vi "Host.vi"() -> ()   [LabVIEW 2019]
uses:
  <vilib>/Bytelabs/ByteTCP/TCP_Class/TCP.lvclass
  TypeDef/TCPMessage.ctl
  <vilib>/Bytelabs/ByteChannelsSetting/ChannelSettingsLib/ChannelsRepos/ChannelsRepoXML/ChannelsRepoXML.lvclass
  TypeDef/listChannel.ctl
  TypeDef/ChannelInfo.ctl
  <vilib>/Bytelabs/ByteChannelsSetting/ChannelSettingsLib/ChannelsClasses/ChannelAnalog/AnalogIn/AnalogIn.lvclass
  ByteGSAPIBase/LimsTestStep/acquisitions.ctl
  ByteGSAPIBase/ByteGSAPIBase.lvclass
  <vilib>/Bytelabs/ByteChannelsSetting/ChannelSettingsLib/ChannelsClasses/ChannelBase/ChannelBase.lvclass
  ByteGSAPIBase/UpdateChannelsList/fields.ctl
  ByteGSAPIBase/TypeDef/Asset.ctl
  ByteGSAPIBase/TypeDef/StepAcquisition.ctl
panel:
  in  "Stop Multiple Log":bool
  out "Map":T1(c390)
  in  "Multiple Log":bool
  in  "Test":T2={"Step Id"=43, "Test Slug"="T0023", "Duration Seconds"=0.0, "Continous?"=FALSE}
  out "error out":errorcluster
  in  "Stop":bool
  out "Results":T3
  in  "Stop Sequence":bool
  out "Status":string
  out "Raws Readings":cluster{"tag":string, "Value":dbl}[](array[cluster])
  in  "Step  Request":bool
  in  "Channel List":T4[](array[typedef])
  in  "Load":bool
  in  "Configuration":bool
  out "Connected?":bool
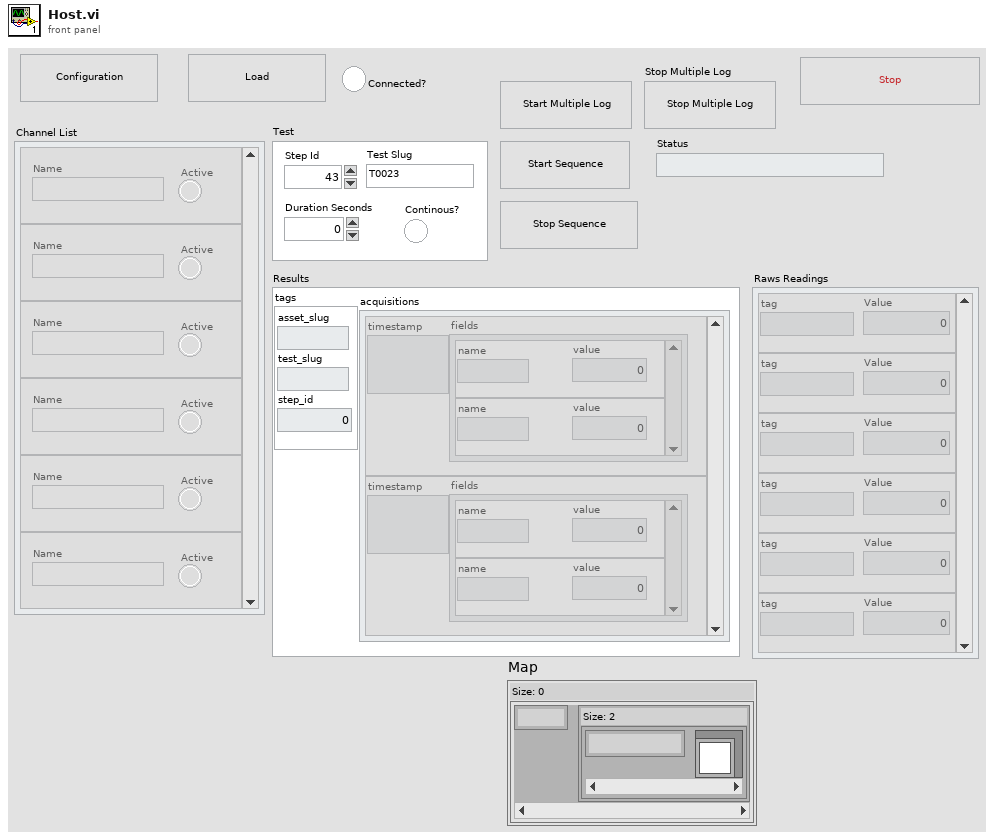
[diagram p1: front panel]
types:
  T1 = map{i32, map{string, refnum<class "ChannelBase.lvclass">}}
  T2 = cluster{"Step Id":u32, "Test Slug":string, "Duration Seconds":dbl, "Continous?":bool}
  T3 = typedef "ByteGSWebAPI.lvlib/ByteGSAPIBase.lvclass/acquisitions.ctl" = cluster{"tags":cluster{"step_id":i32, "test_slug":string, "asset_slug":string}, "acquisitions":cluster{"timestamp":string, "fields":cluster{"name":string, "value":dbl}[]}[]}
  T4 = typedef "listChannel.ctl" = cluster{"Name":string, "Active":bool}
  T5 = typedef "TCPMessage.ctl" = cluster{"Message":string, "Data":variant}
  T6 = cluster{"Event Registration Refnum":refnum<event-registration>, "ChannelsRepoBase out":refnum<class "ChannelsRepoXML.lvclass">, "TCP_Class":refnum<class "TCP.lvclass">, "Data":variant, "Stauts":string, "notifier out":refnum<notifier>}
  T7 = typedef "ChannelInfo.ctl" = cluster{"Tag":string, "HW Resource":string, "Raw":dbl}
  T8 = typedef "ByteGSWebAPI.lvlib/ByteGSAPIBase.lvclass/fields.ctl" = cluster{"asset_slug":string, "fields":string[]}
  T9 = cluster{"Channel List":T4[], "Test":cluster{"Step Id":u32, "Test Slug":string, "Duration Seconds":dbl, "Continous?":bool}}
  T10 = typedef "ByteGSWebAPI.lvlib/ByteGSAPIBase.lvclass/StepAcquisition.ctl" = cluster{"id":i32, "descrizione":string, "prova":cluster{"slug":string}, "assets":T11[], "criterio_accettazione":string, "valore_criterio_accettazione_max":dbl, "valore_criterio_accettazione_min":dbl, "udm_criterio_accettazione":string, "duration_prova":string, "udm_duration_prova":string, "valore_prova":dbl, "ordine":i32, "user":i32, "link_automation":string, "instruction_automation":string, "data_completamento_checklist":timestamp, "outcome":bool, "step_type":string, "channels":string[]}
  T11 = typedef "ByteGSWebAPI.lvlib/ByteGSAPIBase.lvclass/Asset.ctl" = cluster{"descrizione":string, "slug":string, "id":i32}
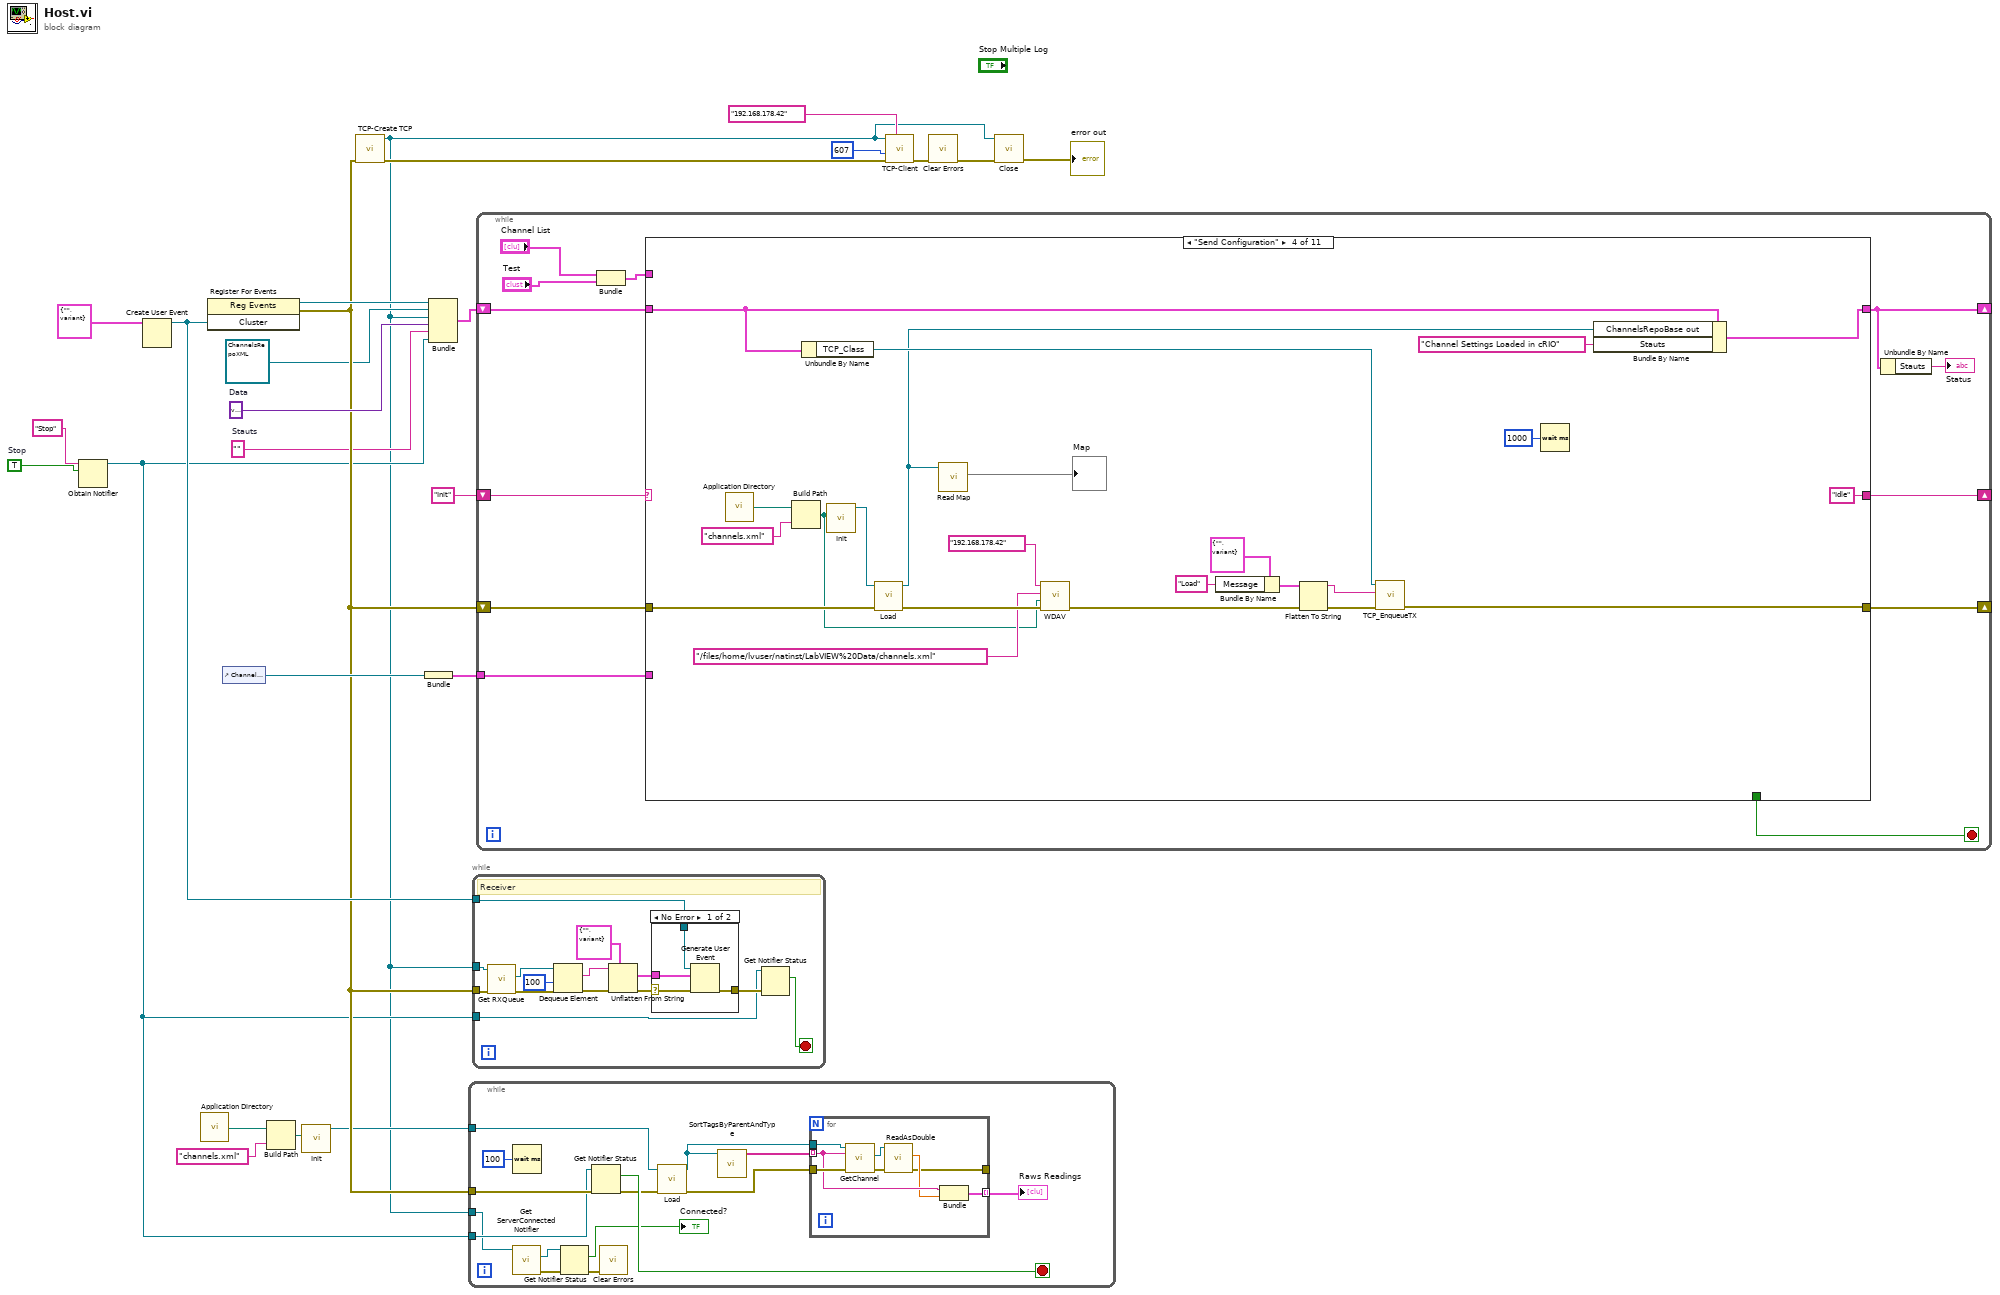
[diagram p0: block diagram]
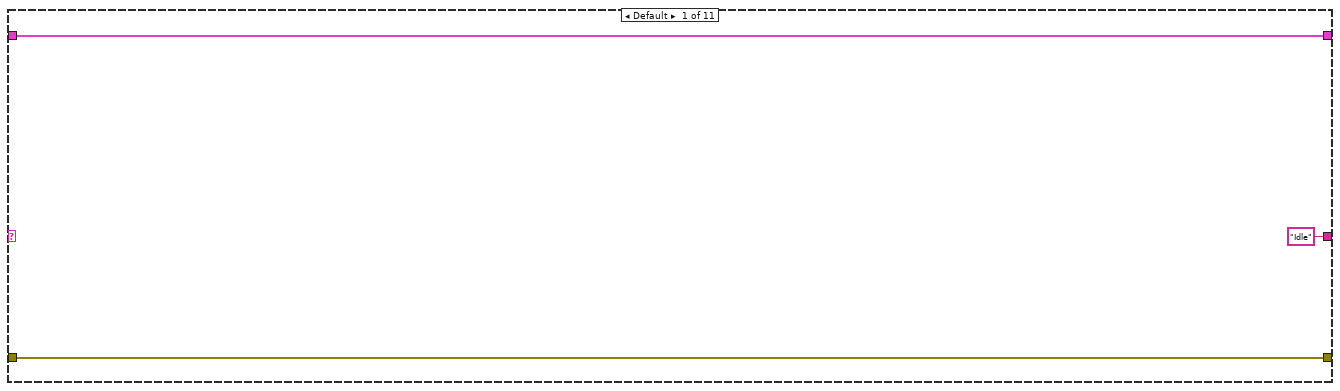
[diagram p2: hidden frame]
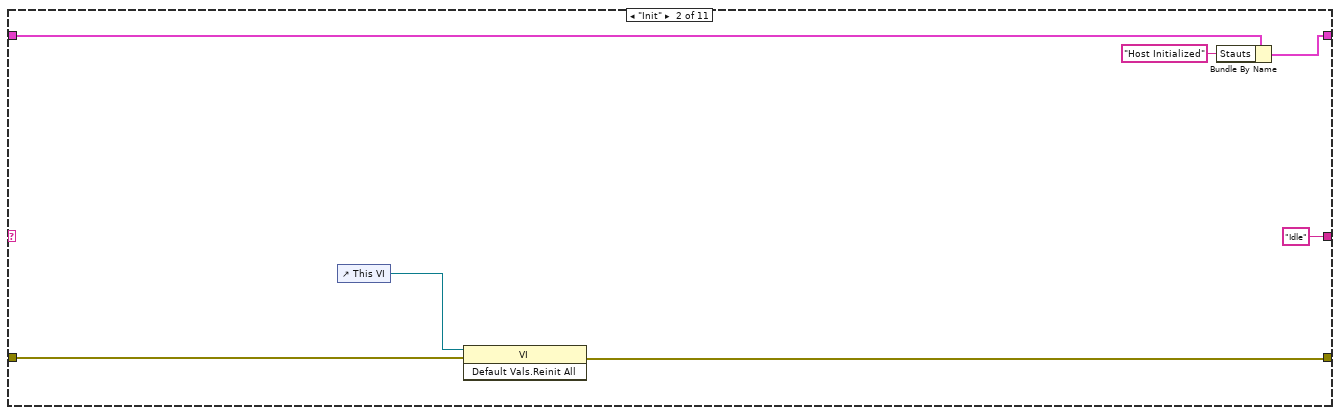
[diagram p3: hidden frame]
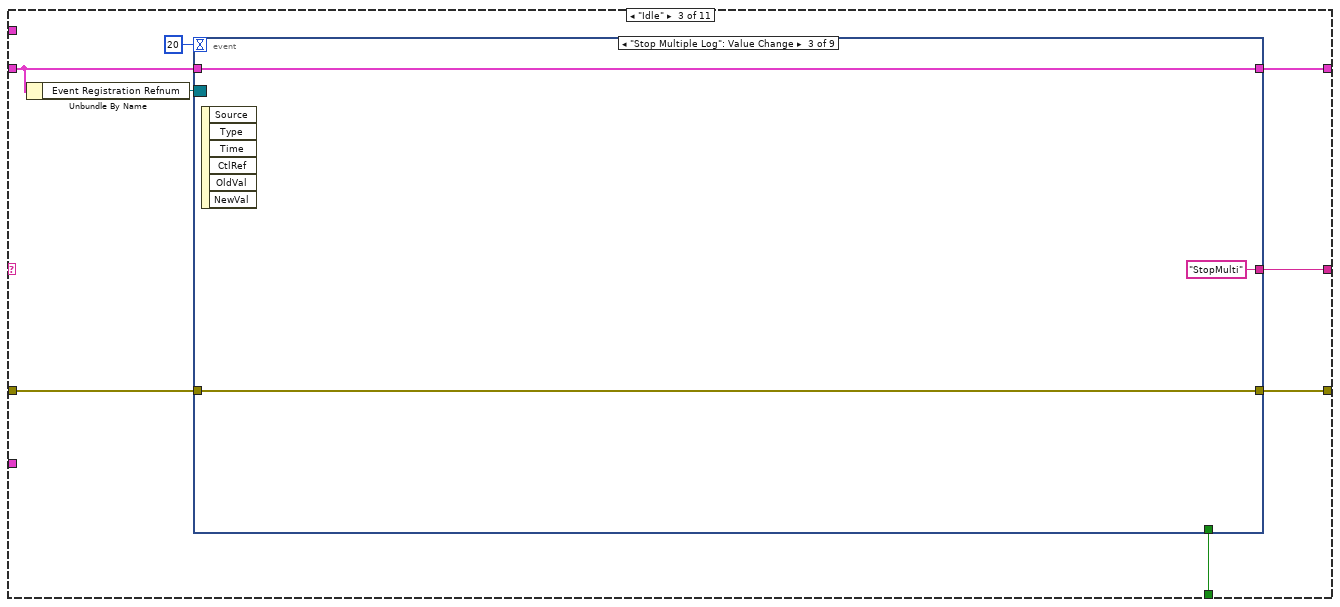
[diagram p4: hidden frame]
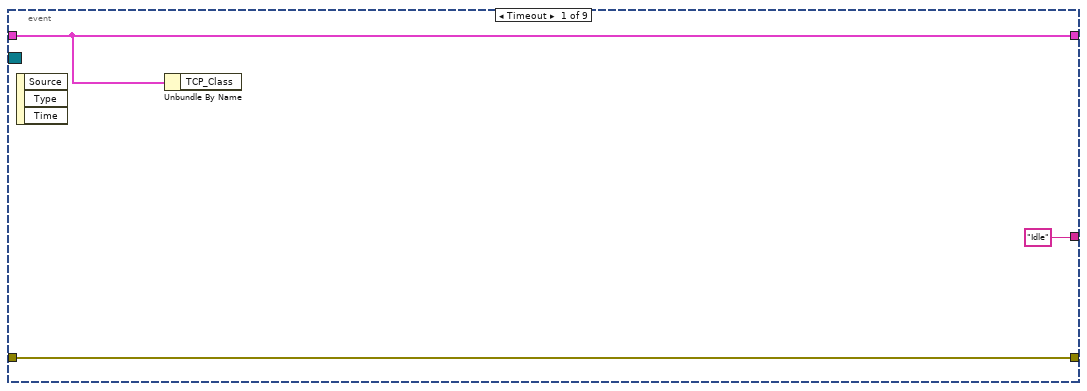
[diagram p5: hidden frame]
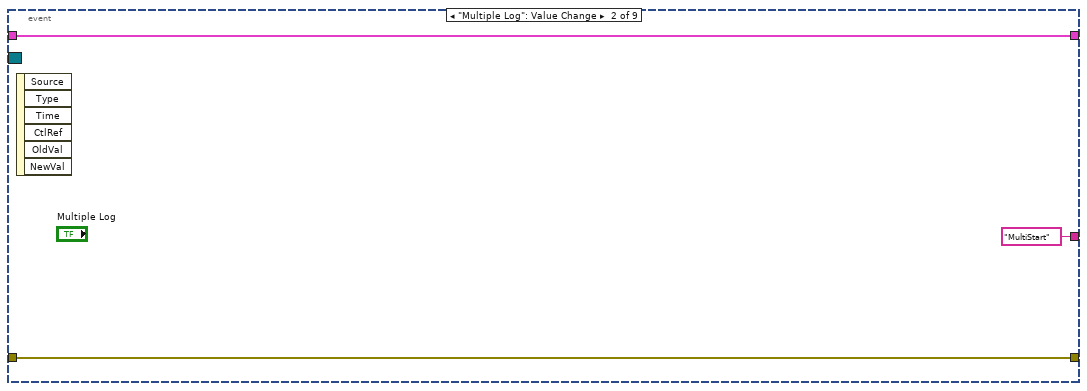
[diagram p6: hidden frame]
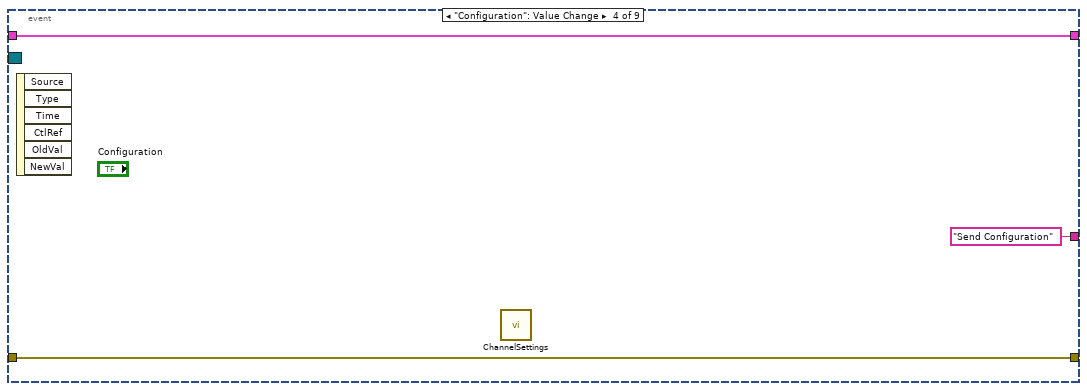
[diagram p7: hidden frame]
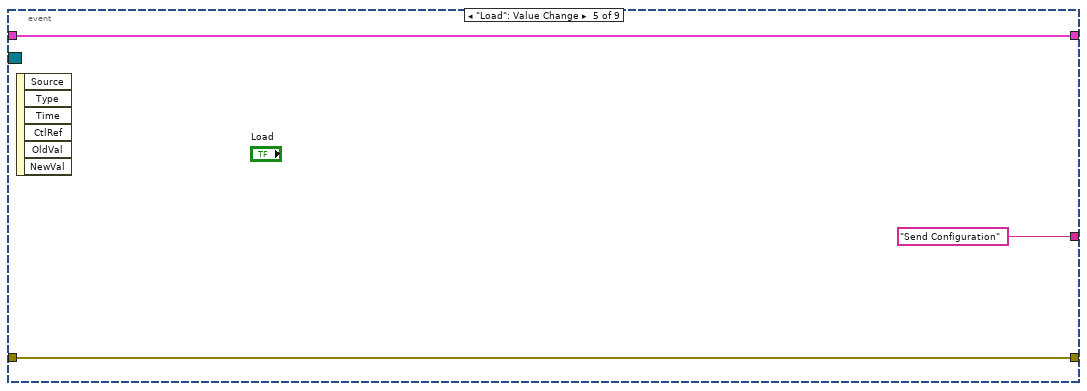
[diagram p8: hidden frame]
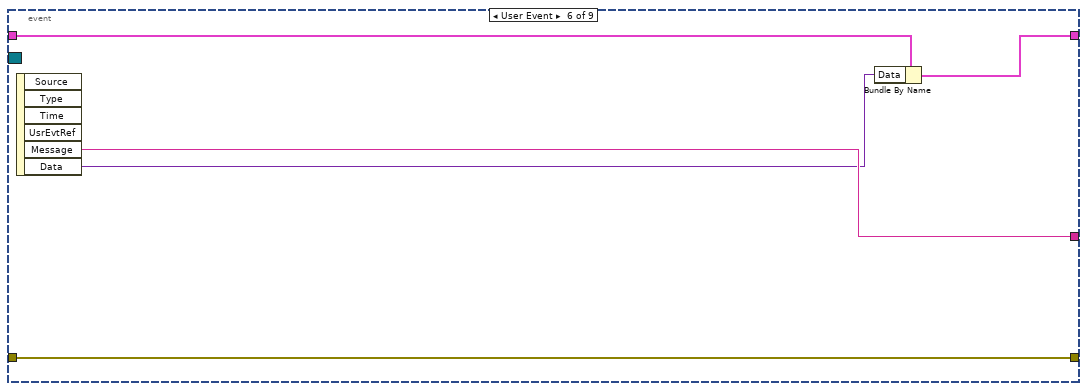
[diagram p9: hidden frame]
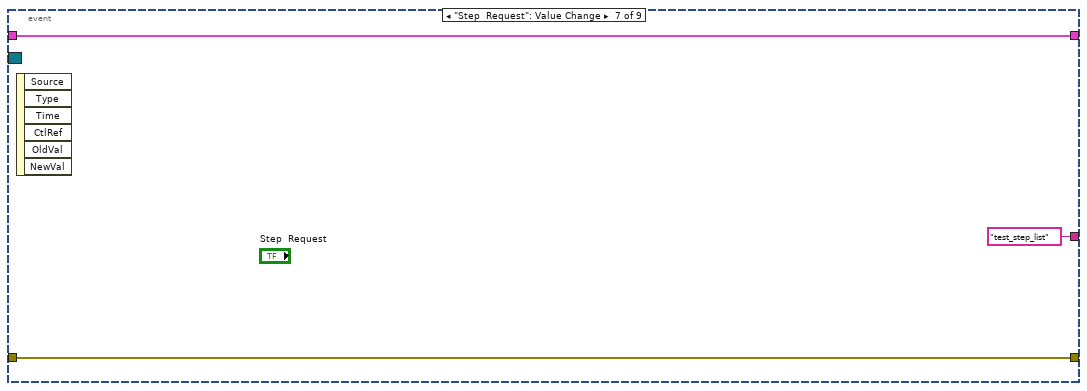
[diagram p10: hidden frame]
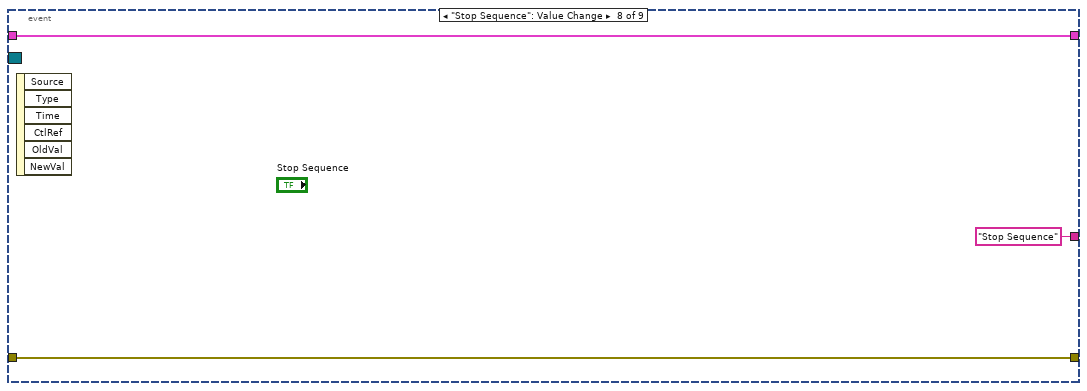
[diagram p11: hidden frame]
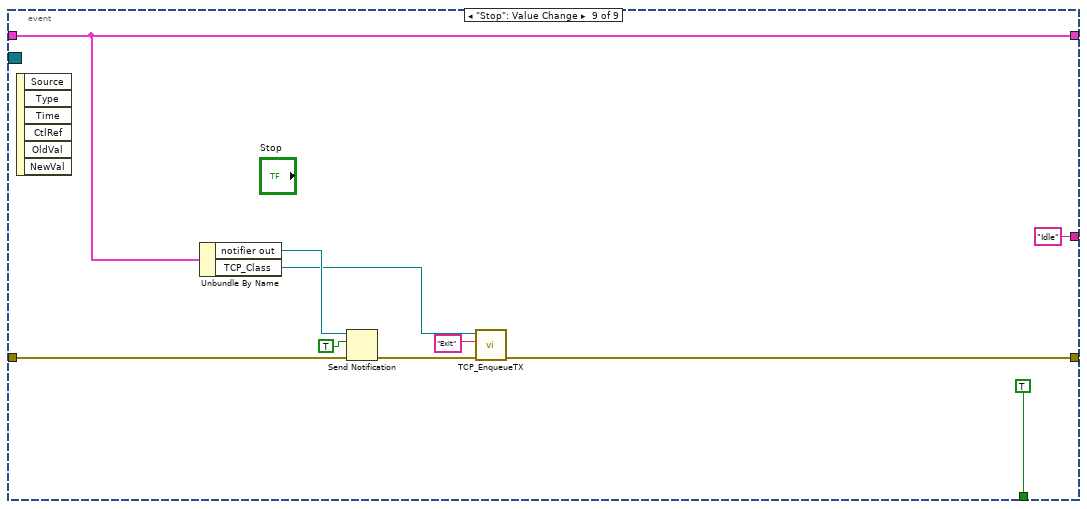
[diagram p12: hidden frame]
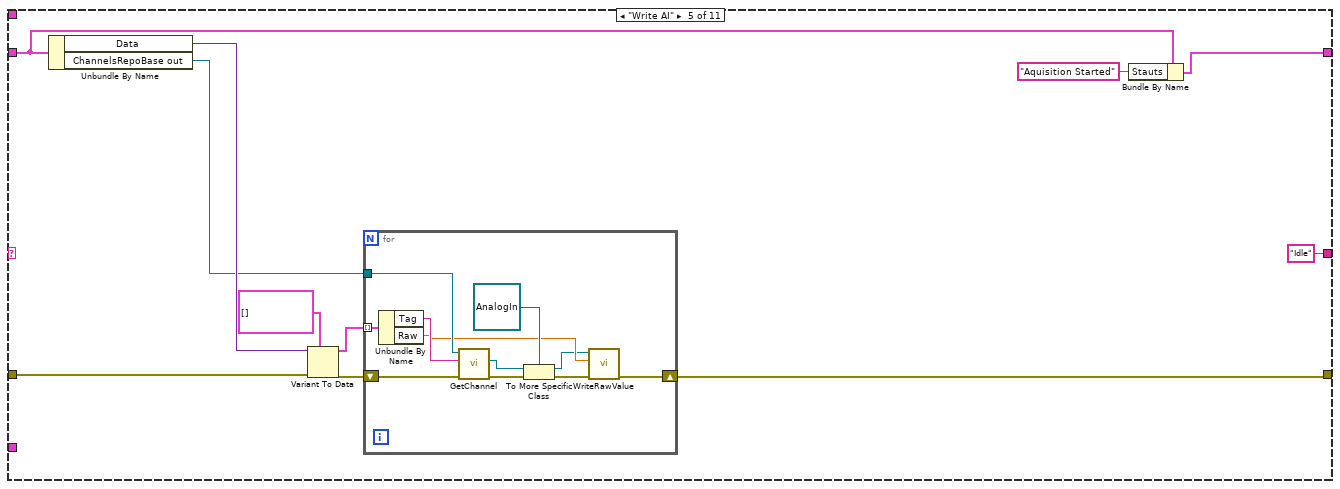
[diagram p13: hidden frame]
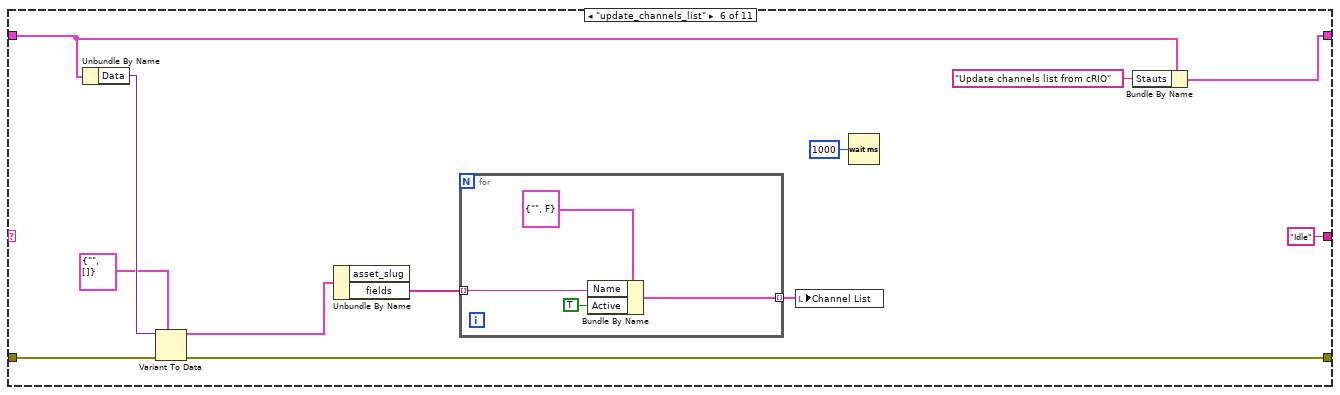
[diagram p14: hidden frame]
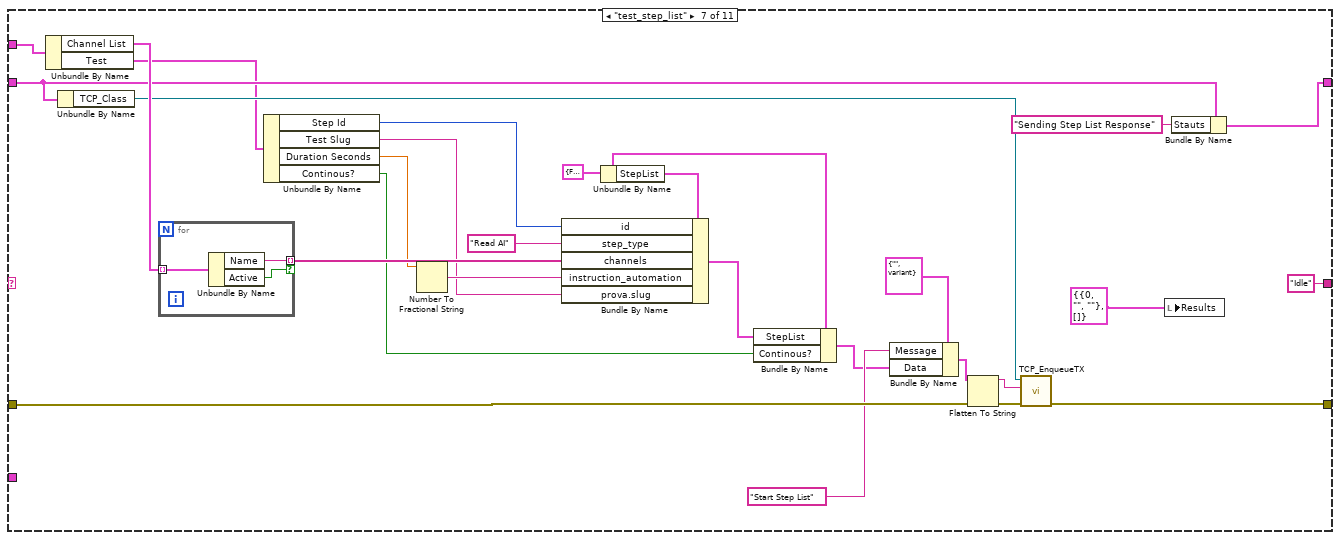
[diagram p15: hidden frame]
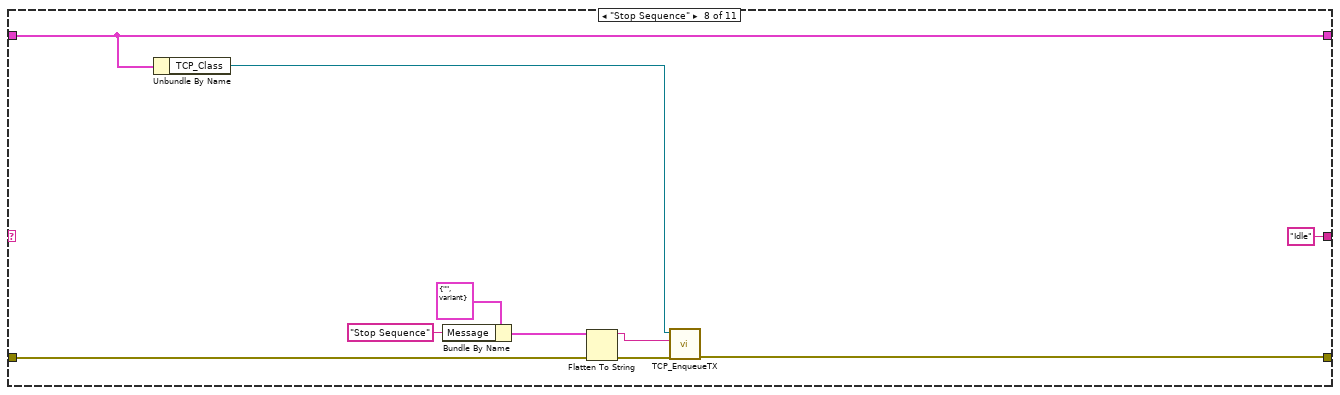
[diagram p16: hidden frame]
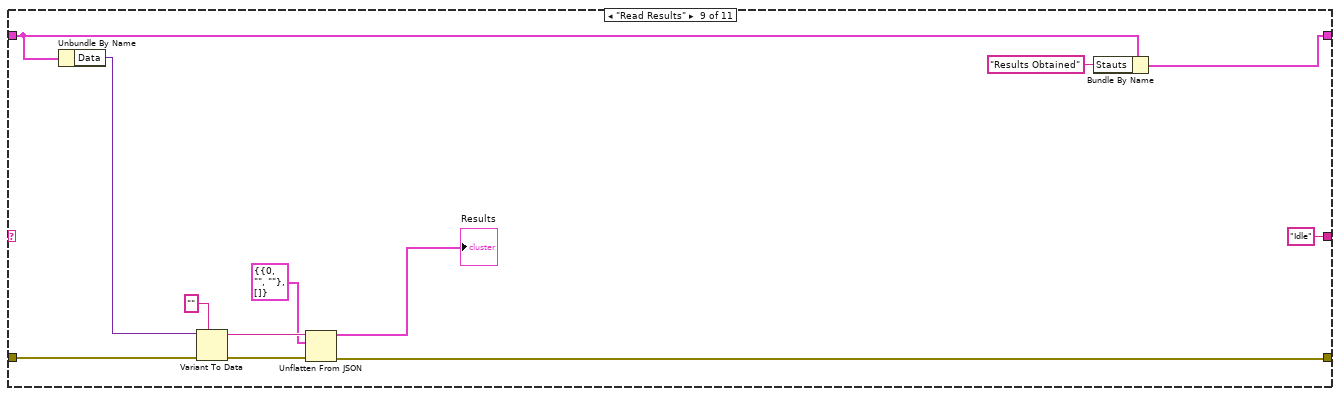
[diagram p17: hidden frame]
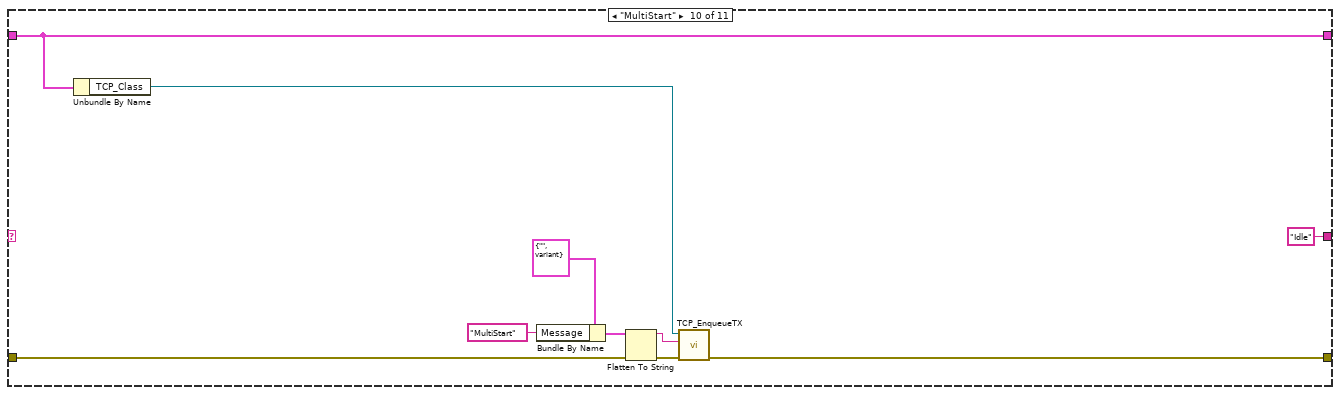
[diagram p18: hidden frame]
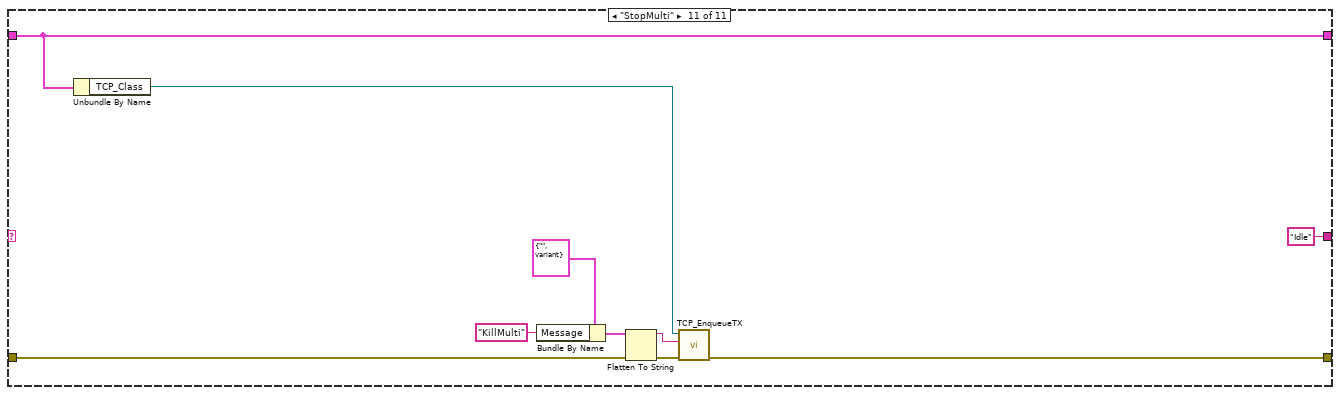
[diagram p19: hidden frame]
diagram:
  w11 = TRUE  # Stop
  w12 = ""  # Stauts
  w17 = variant  # Data
  n1 = Obtain Notifier(name (unnamed)="Stop", notification data type=w11) -> (notifier out=w9:refnum<notifier>)  [unwired: 2 in, 2 out]
  n2 = Create User Event(user event datatype=T5 {"Message"="", "Data"=variant} ("Cluster")) -> (user event=w22:refnum<user-event>)  [unwired: 1 in, 1 out]
  n3 = call <vilib>:"Application Directory.vi"() -> ("Application Directory"=w4:path)
  n4 = register-events(w22) -> (reference out=w21:refnum<event-registration>, error out=w14:errorcluster)  [unwired: 2 in]
  n5 = control-ref of="Channel List"() -> (w16:refnum<vi>)
  n6 = Build Path(base path=w4, name or relative path="channels.xml") -> (appended path=w5:path)
  n7 = call <vilib>:"Init.vi"("XML file path"=w5) -> ("ChannelsRepoXML out"=w2:refnum<class "ChannelsRepoXML.lvclass">)  [unwired: 10 in]
  n8 = call <vilib>:"TCP-Create TCP.vi"("error in (no error)"=w14) -> ("error out"=w23:errorcluster, "TCP_Class"=w1:refnum<class "TCP.lvclass">)  [unwired: 8 in, 1 out]
  n9 = Bundle("Channel List"=w16) -> (w15:cluster{"Channel List":refnum<vi>})  [unwired: 1 in]
  n10 = Bundle("Event Registration Refnum"=w21, "ChannelsRepoBase out"=refnum<class "ChannelsRepoXML.lvclass"> refnum, "TCP_Class"=w1, "Data"=w17, "Stauts"=w12, "notifier out"=w9) -> (w20:T6)  [unwired: 1 in]
  n11 = while {
    tunnel: w14 -> [w36]
    tunnel: w9 -> [w35]
    tunnel: w2 -> [w32]
    tunnel: w1 -> [w27]
    stop <- w34 stop-if-true
    n12 = call-dynamic "Get ServerConnectedNotifier.vi"("TCP in"=w27) -> ("error out"=w29:errorcluster, "IsServerConnected?"=w28:refnum<notifier>)  [unwired: 8 in, 1 out]
    n13 = Wait (ms)(milliseconds to wait=u32 100) -> ()  [unwired: 1 out]
    n14 = Get Notifier Status(notifier=w28, error in (no error)=w29) -> (current notification=→"Connected?":bool, error out=w30:errorcluster)  [unwired: 3 out]
    n15 = Get Notifier Status(notifier=w35, error in (no error)=w36) -> (current notification=w34:bool, error out=w33:errorcluster)  [unwired: 3 out]
    n16 = call <vilib>:"Clear Errors.vi"("error in (no error)"=w30) -> ()  [unwired: 5 in, 2 out]
    n17 = call <vilib>:"Load.vi"("error in (no error)"=w33, "ChannelsRepoBase in"=w32) -> ("error out"=w38:errorcluster, "ChannelsRepoBase out"=w37:refnum<class "ChannelsRepoXML.lvclass">)  [unwired: 7 in, 1 out]
    n18 = call <vilib>:"SortTagsByParentAndType.vi"("ChannelsRepoBase in"=w37) -> ("sorted tags"=w40:string[])  [unwired: 8 in, 2 out]
    n19 = for {
      tunnel: w38 -> [w48]
      tunnel: w40 -> [w45] mode=indexing
      tunnel: [w43] -> w39 mode=indexing
      tunnel: [w42] -> _
      tunnel: w37 -> [w41]
      n20 = call <vilib>:"GetChannel.vi"("error in (no error)"=w48, "tag"=w45, "ChannelsRepoBase in"=w41) -> ("error out"=w47:errorcluster, "channel"=w46:refnum<class "ChannelBase.lvclass">)  [unwired: 5 in, 2 out]
      n21 = call-dynamic "ReadAsDouble.vi"("error in (no error)"=w47, "ChannelBase in"=w46) -> ("error out"=w42:errorcluster, "Value"=w44:dbl)  [unwired: 7 in, 1 out]
      n22 = Bundle("tag"=w45, "Value"=w44) -> (w43:cluster{"tag":string, "Value":dbl})  [unwired: 1 in]
    }
    "Raws Readings" <- w39
  }
  n23 = while {
    tunnel: w1 -> [w57]
    tunnel: w14 -> [w58]
    tunnel: w22 -> [w61]
    tunnel: w9 -> [w51]
    stop <- w50 stop-if-true
    # "Receiver"
    n24 = call-dynamic "Get RXQueue.vi"("error in (no error)"=w58, "TCP in"=w57) -> ("error out"=w56:errorcluster, "RX"=w53:refnum<queue>)  [unwired: 7 in, 1 out]
    n25 = Dequeue Element(queue=w53, timeout in ms (-1)=100, error in (no error)=w56) -> (element=w54:string, error out=w55:errorcluster)  [unwired: 2 out]
    n26 = Unflatten From String(type=T5 {"Message"="", "Data"=variant} ("Cluster"), binary string=w54, error in (no error)=w55) -> (value=w60:T5, error out=w62:errorcluster)  [unwired: 2 in, 1 out]
    n27 = case shown="No Error" w62 {
      selector: w62 -> [w66 _]
      tunnel: w61 -> [w65 _]
      tunnel: w60 -> [w64 _]
      tunnel: [w63 _] -> w52
      frame No Error {
        n28 = Generate User Event(user event=w65, event data cluster=w64, error in=w66) -> (error out=w63:errorcluster)  [unwired: 1 in, 1 out]
      }
      frame Error {
      }
    }
    n29 = Get Notifier Status(notifier=w51, error in (no error)=w52) -> (current notification=w50:bool)  [unwired: 4 out]
  }
  n30 = while {
    shift-right: [w70] -> _
    shift-left: w20 -> [w76]
    shift-right: [w77] -> _
    shift-left: "Init" -> [w78]
    shift-right: [w74] -> _
    shift-left: w14 -> [w75]
    tunnel: w15 -> [w71]
    stop <- w68 stop-if-true
    n31 = Bundle("Channel List"="Channel List", "Test"="Test") -> (w72:T9)  [unwired: 1 in]
    n32 = case shown="\"Send Configuration\"" w78 {
      tunnel: ["Idle" "Idle" w93 "Idle" "Idle" ("Message") "Idle" ("Message") "Idle" ("Message") "Idle" ("Message") "Idle" ("Message") "Idle" ("Message") "Idle" ("Message")] -> w77
      tunnel: w76 -> [w81 w84 w91 w147 w158 w182 w207 w225 w238 w254 w264]
      tunnel: [w81 w82 w92 w146 w157 w180 w206 w225 w236 w254 w264] -> w70
      tunnel: w75 -> [w79 w87 w95 w148 w161 w189 w220 w228 w242 w249 w259]
      tunnel: [w79 w85 w94 w144 w160 w184 w210 w227 w241 w248 w258] -> w74
      tunnel: w72 -> [_ _ _ _ _ _ w218 _ _ _ _]
      tunnel: w71 -> [_ _ _ _ _ _ _ _ _ _ _]
      tunnel: [_ _ w89 _ _ _ _ _ _ _ _] -> w68
      frame Default {
      }
      frame "Init" {
        n33 = control-ref of="This VI"() -> (w86:refnum<vi>)
        n34 = invoke class="VI" method="Default Vals.Reinit All"(reference=w86, error in=w87) -> (error out=w85:errorcluster)  [unwired: 1 in, 2 out]
        n35 = Bundle By Name(cluster=w84, "Stauts"="Host Initialized") -> (w82:T6)
      }
      frame "Idle" {
        n36 = Unbundle By Name(w91) -> ("Event Registration Refnum"=w90:refnum<event-registration>)
        n37 = event shown="[2] \"Stop Multiple Log\": Value Change" {
          selector: w90 -> [_ _ _ _ _ _ _ _ _]
          dyn-events: _ -> [_ _ _ _ _ _ _ _ _]
          timeout: 20 -> [_ _ _ _ _ _ _ _ _]
          tunnel: w91 -> [w98 w102 w105 w108 w111 w115 w119 w121 w130]
          tunnel: w95 -> [w97 w101 w104 w107 w109 w112 w118 w122 w128]
          tunnel: [w97 w101 w104 w107 w109 w112 w118 w122 w125] -> w94
          tunnel: ["Idle" "MultiStart" ("Message") "StopMulti" ("Message") "Send Configuration" "Send Configuration" w116 "test_step_list" ("Message") "Stop Sequence" ("Message") "Idle" ("Message")] -> w93
          tunnel: [w98 w102 w105 w108 w111 w114 w119 w121 w130] -> w92
          tunnel: [_ _ _ _ _ _ _ _ TRUE] -> w89
          event Timeout {
            n38 = event-data() -> ()  [unwired: 1 in, 3 out]
            n39 = Unbundle By Name(w98) -> ()  [unwired: 1 out]
          }
          event "Multiple Log": Value Change {
            n40 = event-data() -> ()  [unwired: 1 in, 6 out]
          }
          event "Stop Multiple Log": Value Change {
            n41 = event-data() -> ()  [unwired: 1 in, 6 out]
          }
          event "Configuration": Value Change {
            n42 = event-data() -> ()  [unwired: 1 in, 6 out]
            n43 = call "ChannelSettings.vi"() -> ()  [unwired: 12 in]
          }
          event "Load": Value Change {
            n44 = event-data() -> ()  [unwired: 1 in, 6 out]
          }
          event User Event {
            n45 = event-data() -> ("Message"=w116:string, "Data"=w113:variant)  [unwired: 1 in, 4 out]
            n46 = Bundle By Name(cluster=w115, "Data"=w113) -> (w114:T6)
          }
          event "Step  Request": Value Change {
            n47 = event-data() -> ()  [unwired: 1 in, 6 out]
          }
          event "Stop Sequence": Value Change {
            n48 = event-data() -> ()  [unwired: 1 in, 6 out]
          }
          event "Stop": Value Change {
            n49 = event-data() -> ()  [unwired: 1 in, 6 out]
            n50 = Unbundle By Name(w130) -> ("notifier out"=w129:refnum<notifier>, "TCP_Class"=w124:refnum<class "TCP.lvclass">)
            n51 = Send Notification(notification=TRUE, notifier=w129, error in (no error)=w128) -> (error out=w126:errorcluster)  [unwired: 1 out]
            n52 = call-dynamic "TCP_EnqueueTX.vi"("error in (no error)"=w126, "Msg to Transmit"="Exit", "TCP in"=w124) -> ("error out"=w125:errorcluster)  [unwired: 7 in, 1 out]
          }
        }
      }
      frame "Send Configuration" {
        n53 = call <vilib>:"Application Directory.vi"() -> ("Application Directory"=w151:path)
        n54 = Build Path(base path=w151, name or relative path="channels.xml") -> (appended path=w135:path)
        n55 = Unbundle By Name(w147) -> ("TCP_Class"=w143:refnum<class "TCP.lvclass">)
        n56 = call <vilib>:"Init.vi"("XML file path"=w135) -> ("ChannelsRepoXML out"=w150:refnum<class "ChannelsRepoXML.lvclass">)  [unwired: 10 in]
        n57 = call <vilib>:"Load.vi"("error in (no error)"=w148, "ChannelsRepoBase in"=w150) -> ("error out"=w139:errorcluster, "ChannelsRepoBase out"=w134:refnum<class "ChannelsRepoXML.lvclass">)  [unwired: 7 in, 1 out]
        n58 = call <vilib>:"Read Map.vi"("ChannelsRepoBase in"=w134) -> ("Map"=→"Map":T1)  [unwired: 9 in, 1 out]
        n59 = call "WDAV.vi"("error in (no error)"=w139, "local file path"=w135, "remote path with slash files"="/files/home/lvuser/natinst/LabVIEW%20Data/channels.xml" ("string"), "target ip"="192.168.178.42") -> ("error out"=w138:errorcluster)  [unwired: 7 in]
        n60 = Bundle By Name(cluster=T5 {"Message"="", "Data"=variant} ("Cluster"), "Message"="Load") -> (w152:T5)
        n61 = Flatten To String(anything=w152, error in (no error)=w138) -> (data string=w142:string, error out=w145:errorcluster)  [unwired: 2 in, 1 out]
        n62 = call-dynamic "TCP_EnqueueTX.vi"("error in (no error)"=w145, "Msg to Transmit"=w142, "TCP in"=w143) -> ("error out"=w144:errorcluster)  [unwired: 7 in, 1 out]
        n63 = Wait (ms)(milliseconds to wait=u32 1000) -> ()  [unwired: 1 out]
        n64 = Bundle By Name(cluster=w147, "ChannelsRepoBase out"=w134, "Stauts"="Channel Settings Loaded in cRIO") -> (w146:T6)
      }
      frame "Write AI" {
        n65 = Unbundle By Name(w158) -> ("Data"=w166:variant, "ChannelsRepoBase out"=w163:refnum<class "ChannelsRepoXML.lvclass">)
        n66 = Variant To Data(error in=w161, type=T7[] [] ("Array"), Variant=w166) -> (data=w162:T7[], error out=w164:errorcluster)
        n67 = for {
          tunnel: w163 -> [w175]
          shift-right: [w169] -> w160
          shift-left: w164 -> [w177]
          tunnel: w162 -> [w167] mode=indexing
          n68 = Unbundle By Name(w167) -> ("Tag"=w176:string, "Raw"=w171:dbl)
          n69 = call <vilib>:"GetChannel.vi"("error in (no error)"=w177, "tag"=w176, "ChannelsRepoBase in"=w175) -> ("error out"=w174:errorcluster, "channel"=w168:refnum<class "ChannelBase.lvclass">)  [unwired: 5 in, 2 out]
          n70 = To More Specific Class(target class=refnum<class "AnalogIn.lvclass"> refnum ("ChannelSettings.lvlib:ChannelsClasses.lvlib:AnalogIn.lvclass"), reference=w168, error in=w174) -> (specific class reference=w170:refnum<class "AnalogIn.lvclass">, error out=w172:errorcluster)
          n71 = call <vilib>:"WriteRawValue.vi"("error in (no error)"=w172, "Raw value"=w171, "AnalogIn in"=w170) -> ("error out"=w169:errorcluster)  [unwired: 7 in, 1 out]
        }
        n72 = Bundle By Name(cluster=w158, "Stauts"="Aquisition Started") -> (w157:T6)
      }
      frame "update_channels_list" {
        n73 = Unbundle By Name(w182) -> ("Data"=w188:variant)
        n74 = Variant To Data(error in=w189, type=T8 {"asset_slug"="", "fields"=[]} ("Channels"), Variant=w188) -> (data=w183:T8, error out=w184:errorcluster)
        n75 = Unbundle By Name(w183) -> ("fields"=w186:string[])  [unwired: 1 out]
        n76 = for {
          tunnel: w186 -> [w192] mode=indexing
          tunnel: [w190] -> w185 mode=indexing
          n77 = Bundle By Name(cluster=T4 {"Name"="", "Active"=FALSE} ("Cluster"), "Name"=w192, "Active"=TRUE) -> (w190:T4)
        }
        n78 = local write "Channel List"(w185) -> ()
        n79 = Wait (ms)(milliseconds to wait=u32 1000) -> ()  [unwired: 1 out]
        n80 = Bundle By Name(cluster=w182, "Stauts"="Update channels list from cRIO") -> (w180:T6)
      }
      frame "test_step_list" {
        w197 = cluster{"Continous?":bool, "StepList":T10} {"Continous?"=FALSE, "StepList"={"id"=0, "descrizione"="", "prova"={"slug"=""}, "assets"=[], "criterio_accettazione"="", "valore_criterio_accettazione_max"=0.0, "valore_criterio_accettazione_min"=0.0, "udm_criterio_accettazione"="", "duration_prova"="", "udm_duration_prova"="", "valore_prova"=0.0, "ordine"=0, "user"=0, "link_automation"="", "instruction_automation"="", "data_completamento_checklist"=timestamp(0 s since 1904-01-01), "outcome"=FALSE, "step_type"="", "channels"=[]}}
        n81 = Unbundle By Name(w218) -> ("Channel List"=w217:T4[], "Test"=w200:T2)
        n82 = Unbundle By Name(w207) -> ("TCP_Class"=w209:refnum<class "TCP.lvclass">)
        n83 = for {
          tunnel: w217 -> [w223] mode=indexing
          tunnel: [w222] -> w216 mode=indexing if=w221
          n84 = Unbundle By Name(w223) -> ("Name"=w222:string, "Active"=w221:bool)
        }
        n85 = Unbundle By Name(w200) -> ("Step Id"=w202:u32, "Test Slug"=w201:string, "Duration Seconds"=w199:dbl, "Continous?"=w195:bool)
        n86 = Number To Fractional String(number=w199) -> (F-format string=w204:string)  [unwired: 3 in]
        n87 = Unbundle By Name(w197) -> ("StepList"=w198:T10)
        n88 = Bundle By Name(cluster=w198, "id"=w202, "step_type"="Read AI", "channels"=w216, "instruction_automation"=w204, "prova.slug"=w201) -> (w196:T10)
        n89 = Bundle By Name(cluster=w197, "StepList"=w196, "Continous?"=w195) -> (w194:cluster{"Continous?":bool, "StepList":T10})
        n90 = Bundle By Name(cluster=T5 {"Message"="", "Data"=variant} ("Cluster"), "Message"="Start Step List", "Data"=w194) -> (w212:T5)
        n91 = Flatten To String(anything=w212, error in (no error)=w220) -> (data string=w211:string, error out=w213:errorcluster)  [unwired: 2 in, 1 out]
        n92 = call-dynamic "TCP_EnqueueTX.vi"("error in (no error)"=w213, "Msg to Transmit"=w211, "TCP in"=w209) -> ("error out"=w210:errorcluster)  [unwired: 7 in, 1 out]
        n93 = local write "Results"(T3 {"tags"={"step_id"=0, "test_slug"="", "asset_slug"=""}, "acquisitions"=[]}) -> ()
        n94 = Bundle By Name(cluster=w207, "Stauts"="Sending Step List Response") -> (w206:T6)
      }
      frame "Stop Sequence" {
        n95 = Unbundle By Name(w225) -> ("TCP_Class"=w224:refnum<class "TCP.lvclass">)
        n96 = Bundle By Name(cluster=T5 {"Message"="", "Data"=variant} ("Cluster"), "Message"="Stop Sequence") -> (w231:T5)
        n97 = Flatten To String(anything=w231, error in (no error)=w228) -> (data string=w229:string, error out=w230:errorcluster)  [unwired: 2 in, 1 out]
        n98 = call-dynamic "TCP_EnqueueTX.vi"("error in (no error)"=w230, "Msg to Transmit"=w229, "TCP in"=w224) -> ("error out"=w227:errorcluster)  [unwired: 7 in, 1 out]
      }
      frame "Read Results" {
        n99 = Unbundle By Name(w238) -> ("Data"=w240:variant)
        n100 = Variant To Data(error in=w242, type="", Variant=w240) -> (data=w243:string, error out=w245:errorcluster)
        n101 = Unflatten From JSON(JSON string=w243, type and defaults=T3 {"tags"={"step_id"=0, "test_slug"="", "asset_slug"=""}, "acquisitions"=[]}, error in (no error)=w245) -> (value=→"Results":T3, error out=w241:errorcluster)  [unwired: 4 in]
        n102 = Bundle By Name(cluster=w238, "Stauts"="Results Obtained") -> (w236:T6)
      }
      frame "MultiStart" {
        n103 = Unbundle By Name(w254) -> ("TCP_Class"=w247:refnum<class "TCP.lvclass">)
        n104 = Bundle By Name(cluster=T5 {"Message"="", "Data"=variant} ("Cluster"), "Message"="MultiStart") -> (w251:T5)
        n105 = Flatten To String(anything=w251, error in (no error)=w249) -> (data string=w250:string, error out=w252:errorcluster)  [unwired: 2 in, 1 out]
        n106 = call-dynamic "TCP_EnqueueTX.vi"("error in (no error)"=w252, "Msg to Transmit"=w250, "TCP in"=w247) -> ("error out"=w248:errorcluster)  [unwired: 7 in, 1 out]
      }
      frame "StopMulti" {
        n107 = Unbundle By Name(w264) -> ("TCP_Class"=w257:refnum<class "TCP.lvclass">)
        n108 = Bundle By Name(cluster=T5 {"Message"="", "Data"=variant} ("Cluster"), "Message"="KillMulti") -> (w261:T5)
        n109 = Flatten To String(anything=w261, error in (no error)=w259) -> (data string=w260:string, error out=w262:errorcluster)  [unwired: 2 in, 1 out]
        n110 = call-dynamic "TCP_EnqueueTX.vi"("error in (no error)"=w262, "Msg to Transmit"=w260, "TCP in"=w257) -> ("error out"=w258:errorcluster)  [unwired: 7 in, 1 out]
      }
    }
    n111 = Unbundle By Name(w70) -> ("Stauts"=→"Status":string)
  }
  n112 = call <vilib>:"TCP-Client.vi"("IP address"="192.168.178.42", "error in (no error)"=w23, "TXport"=u16 607 ("port"), "TCP.lvclass"=w1) -> ("error out"=w7:errorcluster)  [unwired: 7 in]
  n113 = call <vilib>:"Clear Errors.vi"("error in (no error)"=w7) -> ("error out"=w6:errorcluster)  [unwired: 5 in, 1 out]
  n114 = call-dynamic "Close.vi"("error in (no error)"=w6, "TCP in"=w1) -> ("error out"=→"error out":errorcluster)  [unwired: 5 in, 4 out]
